vi "fake tool confirm.vi"() -> (0 "error out":errorcluster, 3 "outcome":string)   [LabVIEW 2020, in "MCP Server tests.lvlib"]
doc: "Fake tool to test elicitation. It asks the user \"Run the fake action?\" with Confirm With User.vi (key confirm_action) and reports on outcome which path it took: pending (first run, returns at once without doing anything), confirmed, declined or not supported (legacy client or no elicitation capability)."
uses:
  MCP Server tests.lvlib
  src/MCP Server/MCP Server.lvlib
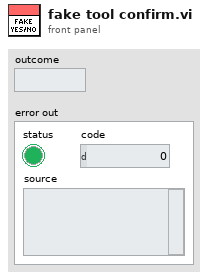
[diagram p1: front panel]
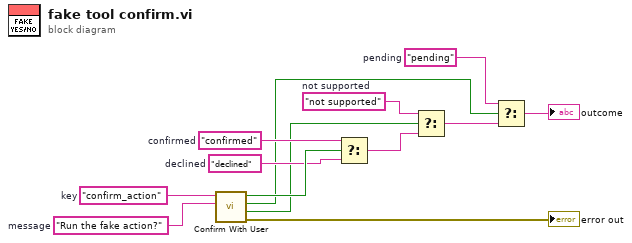
[diagram p0: block diagram]
diagram:
  w5 = "pending"  # pending
  w8 = "not supported"  # not supported
  w9 = "declined"  # declined
  w11 = "confirmed"  # confirmed
  w12 = "Run the fake action?"  # message
  w13 = "confirm_action"  # key
  n1 = call "Confirm With User.vi"("message"=w12, "key"=w13) -> ("error out"=→"error out":errorcluster, "not supported?"=w7:bool, "pending?"=w4:bool, "confirmed?"=w10:bool)  [unwired: 6 in]
  n2 = Select(t=w11, s=w10, f=w9) -> (s? t:f=w6:string)
  n3 = Select(t=w8, s=w7, f=w6) -> (s? t:f=w3:string)
  n4 = Select(t=w5, s=w4, f=w3) -> (s? t:f=→"outcome":string)
